vi "Event QueryIfComplete.vi"(8 "error in (no error)":errorcluster, 11 "Event in":refnum<class "Event.lvclass">) -> (0 "error out":errorcluster, 2 "IsComplete?":bool, 3 "Event out":refnum<class "Event.lvclass">)   [LabVIEW 2020, in "OpenLvVision_OpenCv.lvlib" / "Cuda.lvlib" / "Event.lvclass"]
doc: "Performs a non-blocking check to see if the event has triggered yet."
uses:
  Event.lvclass
  C:/Users/lukas/Downloads/OpenLvVision_OpenCv/SourceCode/LabView/OpenLvVision_OpenCv/_LvHelpers/EdvrObject/EdvrObject.lvclass
  _LvHelpers/EdvrObject/EdvrObject.lvclass/EdvrObject.ctl
  OpenLvVision_OpenCv.lvlib
  _LvHelpers/EdvrObject/EdvrObject.lvclass
  <vilib>/Utility/error.llb/Error Cluster From Error Code.vi
  <vilib>/ErrorRing/Error Ring.xnode
  Dlls/OlvOpenCvWrapper.dll
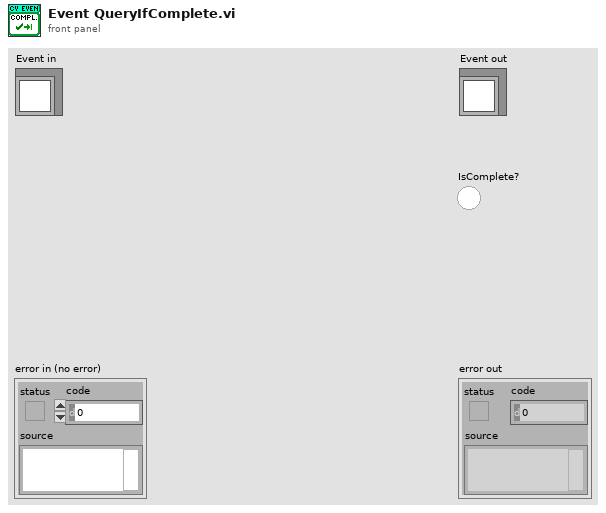
[diagram p1: front panel]
types:
  T1 = typedef "OpenLvVision_OpenCv.lvlib/EdvrObject.lvclass/Edvr.ctl" = refnum<data-value>
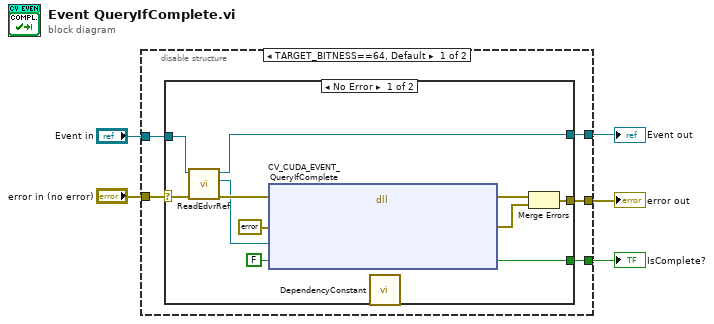
[diagram p0: block diagram]
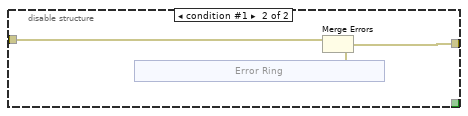
[diagram p3: hidden frame]
diagram:
  n1 = disable-structure shown="TARGET_BITNESS==64, Default" {
    disable-tunnel: "error in (no error)" -> [w7 w25]
    disable-tunnel: [w10 w26] -> w5
    disable-tunnel: [w9 _] -> w4
    disable-tunnel: "Event in" -> [w8 _]
    disable-tunnel: [w6 _] -> w1
    frame condition #0 (active) {
      n2 = case shown="No Error" w7 {
        selector: w7 -> [w15 w23]
        tunnel: [w17 w23] -> w10
        tunnel: [w18 w22] -> w9
        tunnel: w8 -> [w16 w22]
        tunnel: [w11 _] -> w6
        frame No Error {
          n3 = call "ReadEdvrRef.vi"("error in (no error)"=w15, "EdvrObject in"=w16) -> ("error out"=w20:errorcluster, "Edvr"=w19:T1, "EdvrObject out"=w18:refnum<class "Event.lvclass">)  [unwired: 7 in]
          n4 = dll-call lib="C:/Users/lukas/Downloads/OpenLvVision_OpenCv/SourceCode/LabView/OpenLvVision_OpenCv/Dlls/OlvOpenCvWrapper.dll" fn="CV_CUDA_EVENT_QueryIfComplete"(error in=w20, "Error"=errorcluster {"status"=FALSE, "code"=0, "source"=""} ("error out"), "eventEdvrRef"=w19, "result"=FALSE) -> (error out=w13:errorcluster, "Error"=w14:errorcluster, "result"=w11:bool)  [unwired: 4 in, 1 out]
          n5 = call "DependencyConstant.vi"() -> ()  [unwired: 12 in]
          n6 = Merge Errors(w13, w14) -> (w17:errorcluster)
        }
        frame Error {
        }
      }
    }
    frame condition #1 {
      n7 = xnode "Error Ring"() -> ("error out"=w24:errorcluster)
      n8 = Merge Errors(w25, w24) -> (w26:errorcluster)
    }
  }
  "error out" <- w5
  "Event out" <- w4
  "IsComplete?" <- w1
